vi "Select Point.vi"(8 "error in (no error)":errorcluster caption="错误输入（无错误）", 11 "Data Viewer 输入":refnum<class "Data Viewer.lvclass">) -> (0 "error out":errorcluster caption="错误输出", 3 "Data Viewer 输出":refnum<class "Data Viewer.lvclass">)   [LabVIEW 2020, in "Data Viewer.lvlib" / "Data Viewer.lvclass"]
uses:
  Data Viewer.lvclass
  Data Viewer.lvclass/Data Viewer.ctl
  NI/20_cRIO/Axis Controller V4/Axis Controller UI/Libraries/Data Save/Linear Measurement Panel/Point.ctl
  NI/20_cRIO/Axis Controller V4/Axis Controller UI/Libraries/Data Save/Linear Measurement Panel/Linear Measurement Panel.lvlib
panel:
  out "Curve Clip":cluster{dbl[], dbl[]}
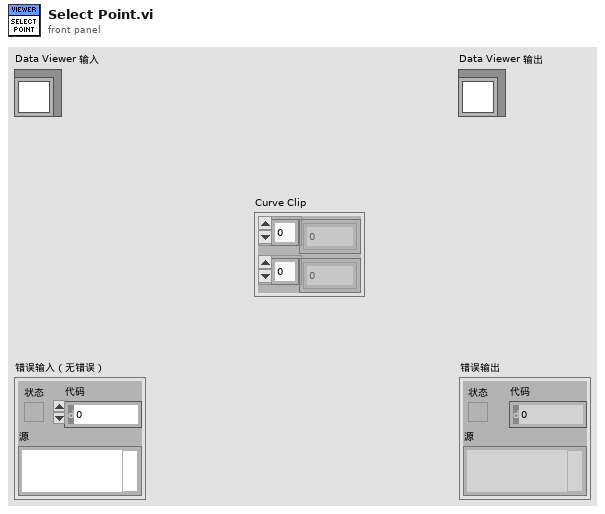
[diagram p1: front panel]
types:
  T1 = typedef "Data Save.lvlib/Linear Measurement Panel.lvlib/Point.ctl" = cluster{"Curve":i32, "X":dbl, "Y":dbl}
  T2 = cluster{"Curve":i32, "Point":cluster{"X":dbl, "Y":dbl}}
  T3 = typedef "LVPoint32TypeDef.ctl" = cluster{"Horizontal":i32, "Vertical":i32}
  T4 = typedef "LVBoundsTypeDef.ctl" = cluster{"Width":u32, "Height":u32}
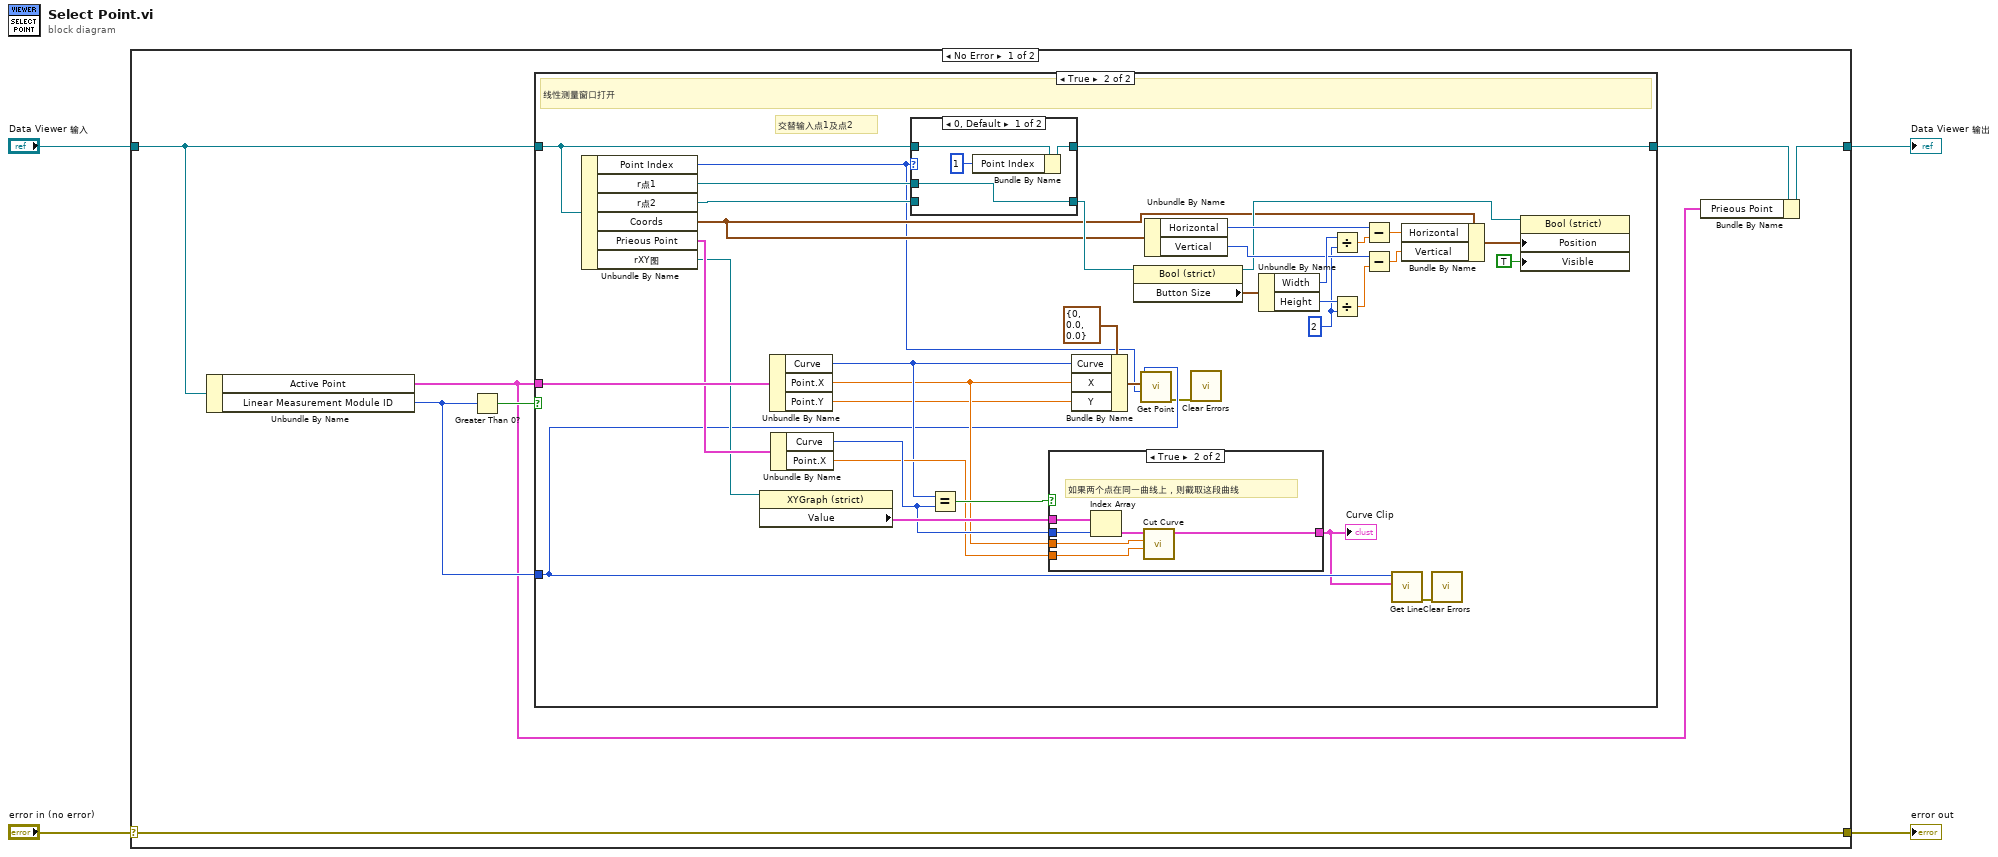
[diagram p0: block diagram]
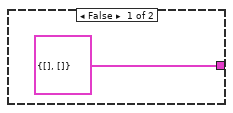
[diagram p3: hidden frame]
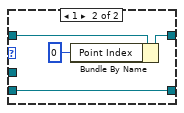
[diagram p4: hidden frame]
diagram:
  n1 = case shown="No Error" "error in (no error)" {
    selector: "error in (no error)" -> [w11 w65]
    tunnel: [w11 w65] -> w3
    tunnel: [w6 w64] -> w1
    tunnel: "Data Viewer 输入" -> [w8 w64]
    frame No Error {
      n2 = Unbundle By Name(w8) -> ("Active Point"=w5:T2, "Linear Measurement Module ID"=w9:i32)
      n3 = Greater Than 0?(x=w9) -> (x > 0?=w10:bool)
      n4 = case shown="True" w10 {
        tunnel: [w12 w48] -> w7
        tunnel: w8 -> [w12 w47]
        tunnel: w9 -> [_ w16]
        tunnel: w5 -> [_ w26]
        frame False {
        }
        frame True {
          w33 = u32 2 ("y")
          # "交替输入点1及点2"
          # "线性测量窗口打开"
          n5 = Unbundle By Name(w47) -> ("Point Index"=w27:i32, "r点1"=w46:refnum<vi>, "r点2"=w45:refnum<vi>, "Coords"=w30:T3, "Prieous Point"=w18:T2, "rXY图"=w17:refnum<vi>)
          n6 = property class="XYGraph (strict)"(reference=w17) -> ("Value"=w25:cluster{dbl[], dbl[]}[])  [unwired: 1 in, 2 out]
          n7 = Unbundle By Name(w26) -> ("Curve"=w21:i32, "Point.X"=w20:dbl, "Point.Y"=w19:dbl)
          n8 = Unbundle By Name(w18) -> ("Curve"=w23:i32, "Point.X"=w22:dbl)
          n9 = case shown="0, Default" w27 {
            tunnel: [w58 w62] -> w48
            tunnel: w47 -> [w59 w63]
            tunnel: w46 -> [w56 _]
            tunnel: w45 -> [_ w60]
            tunnel: [w56 w60] -> w31
            frame 0, Default {
              n10 = Bundle By Name(cluster=w59, "Point Index"=1) -> (w58:refnum<class "Data Viewer.lvclass">)
            }
            frame 1 {
              n11 = Bundle By Name(cluster=w63, "Point Index"=0) -> (w62:refnum<class "Data Viewer.lvclass">)
            }
          }
          n12 = Equal?(x=w21, y=w23) -> (x = y?=w24:bool)
          n13 = case shown="True" w24 {
            tunnel: w25 -> [_ w55]
            tunnel: w23 -> [_ w54]
            tunnel: w20 -> [_ w52]
            tunnel: w22 -> [_ w51]
            tunnel: [cluster{dbl[], dbl[]} {[], []} ("Cut Curve") w50] -> w13
            frame False {
            }
            frame True {
              # "如果两个点在同一曲线上，则截取这段曲线"
              n14 = Index Array(array=w55, index=w54) -> (element=w53:cluster{dbl[], dbl[]})
              n15 = call "Cut Curve.vi"("X2"=w51, "X1"=w52, "Curve"=w53) -> ("Cut Curve"=w50:cluster{dbl[], dbl[]})  [unwired: 8 in]
            }
          }
          "Curve Clip" <- w13
          n16 = Bundle By Name(cluster=T1 {"Curve"=0, "X"=0.0, "Y"=0.0} ("Point"), "Curve"=w21, "X"=w20, "Y"=w19) -> (w29:T1)
          n17 = property class="Bool (strict)"(reference=w31) -> (reference out=w34:refnum<vi>, "Button Size"=w44:T4)  [unwired: 1 in, 1 out]
          n18 = call "Get Point.vi"("Point Index"=w27, "Point"=w29, "Module ID"=w16) -> ("error out"=w15:errorcluster)  [unwired: 8 in]
          n19 = Unbundle By Name(w30) -> ("Horizontal"=w43:i32, "Vertical"=w39:i32)
          n20 = call <vilib>:"Clear Errors.vi"("error in (no error)"=w15) -> ()  [unwired: 5 in, 2 out]
          n21 = Unbundle By Name(w44) -> ("Width"=w42:u32, "Height"=w40:u32)
          n22 = Divide(x=w42, y=w33) -> (x/y=w41:dbl)
          n23 = Divide(x=w40, y=w33) -> (x/y=w38:dbl)
          n24 = Subtract(x=w43, y=w41) -> (x-y=w37:dbl)
          n25 = Subtract(x=w39, y=w38) -> (x-y=w36:dbl)
          n26 = call "Get Line.vi"("Curve Clip"=w13, "Module ID"=w16) -> ("error out"=w14:errorcluster)  [unwired: 9 in]
          n27 = Bundle By Name(cluster=w30, "Horizontal"=w37, "Vertical"=w36) -> (w35:T3)
          n28 = call <vilib>:"Clear Errors.vi"("error in (no error)"=w14) -> ()  [unwired: 5 in, 2 out]
          n29 = property class="Bool (strict)"(reference=w34, "Position"=w35, "Visible"=TRUE ("可见")) -> ()  [unwired: 1 in, 2 out]
        }
      }
      n30 = Bundle By Name(cluster=w7, "Prieous Point"=w5) -> (w6:refnum<class "Data Viewer.lvclass">)
    }
    frame Error {
    }
  }
  "error out" <- w3
  "Data Viewer 输出" <- w1
